vi "Migrate Measurement Dependencies.vi"(0 "project path":path, 1 "init":T1[](array[typedef]), 5 "measurement path":path, 7 "dependencies path":path[](array[path]), 9 "plug-in name":string, 11 "error in":errorcluster) -> (4 "project reference":refnum<vi>, 6 "measurement core reference":refnum<vi>, 8 "outside items":string[](array[string]), 10 "copied standalone VIs":cluster{"Lib path":path, "VI path":path}[](array[cluster]), 15 "error out":errorcluster)   [LabVIEW 2021, in "Multiple Converter.lvlib"]
uses:
  Multiple Converter.lvlib
  TypeDefs/Library Info.ctl
  Path Functions/Path Functions.lvlib
  Converter Reusables/Converter Reusables.lvlib
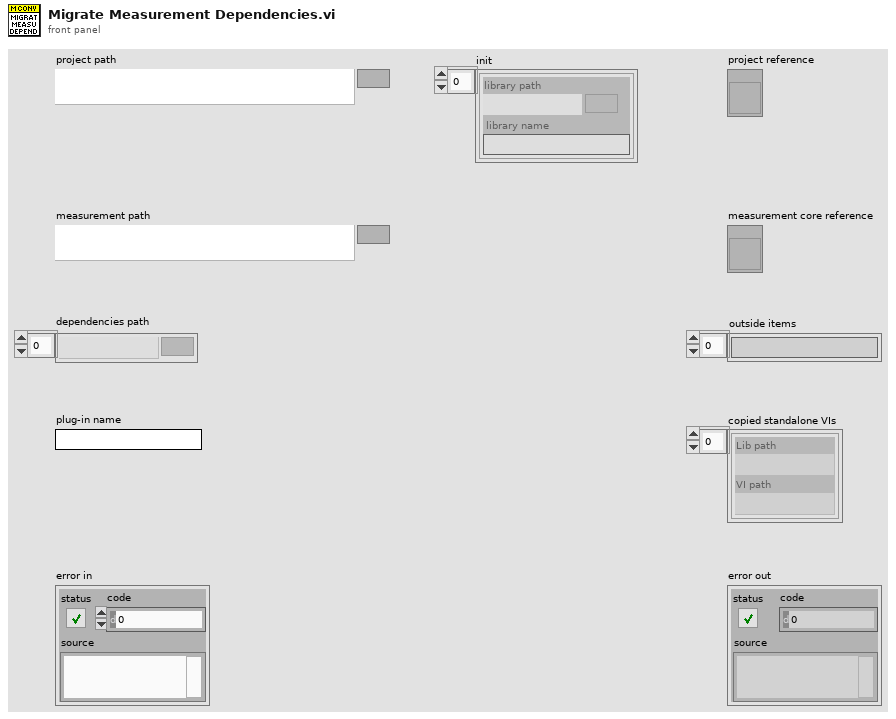
[diagram p1: front panel]
types:
  T1 = typedef "Multiple Converter.lvlib/Library Info.ctl" = cluster{"library path":path, "library name":string}
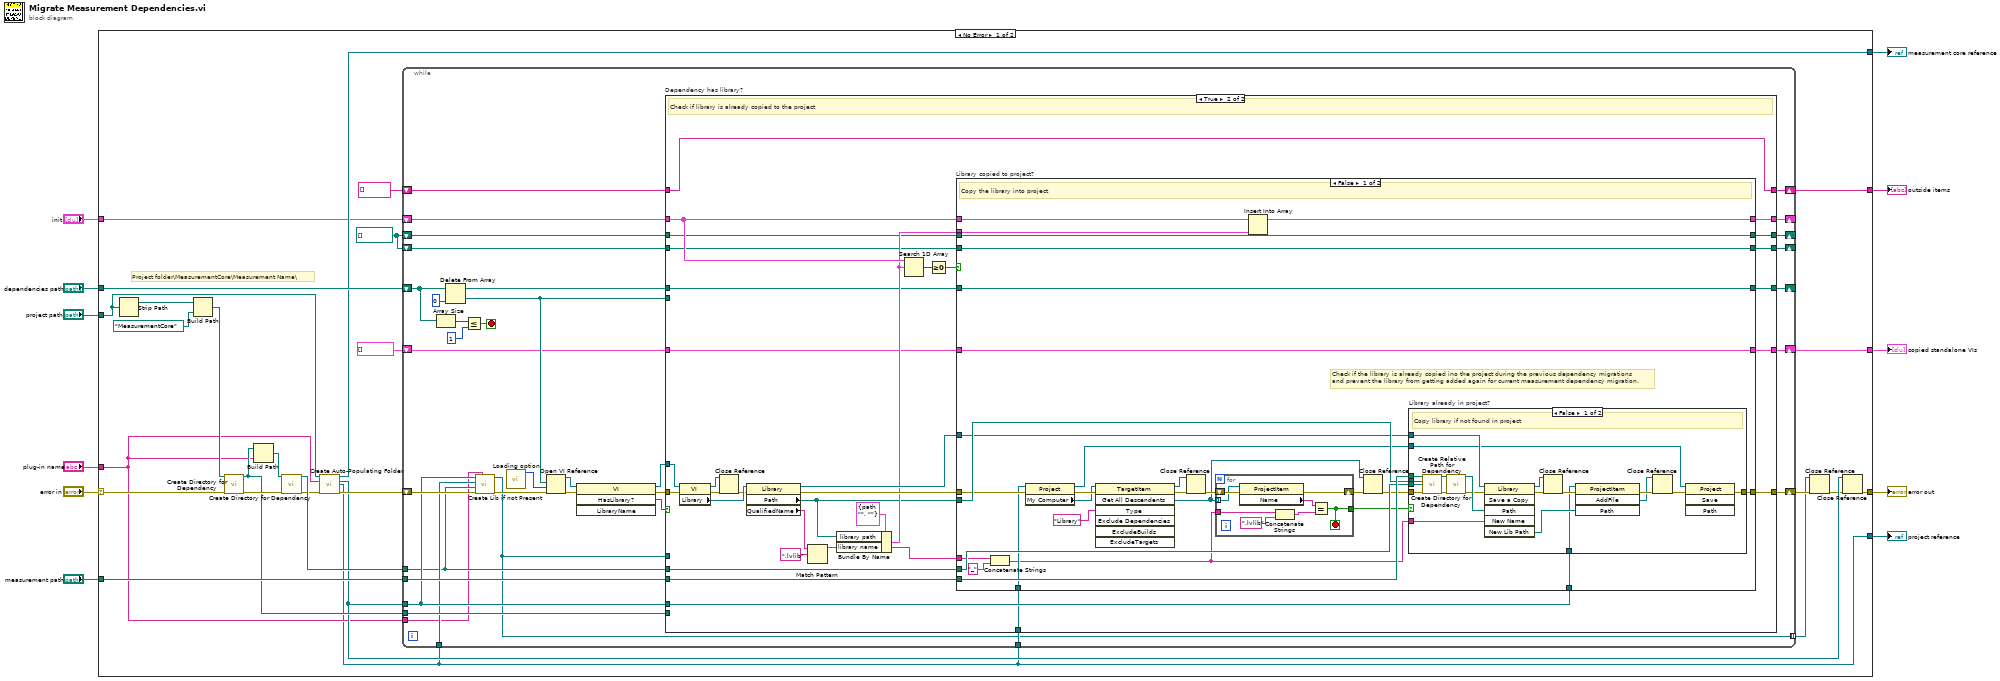
[diagram p0: block diagram]
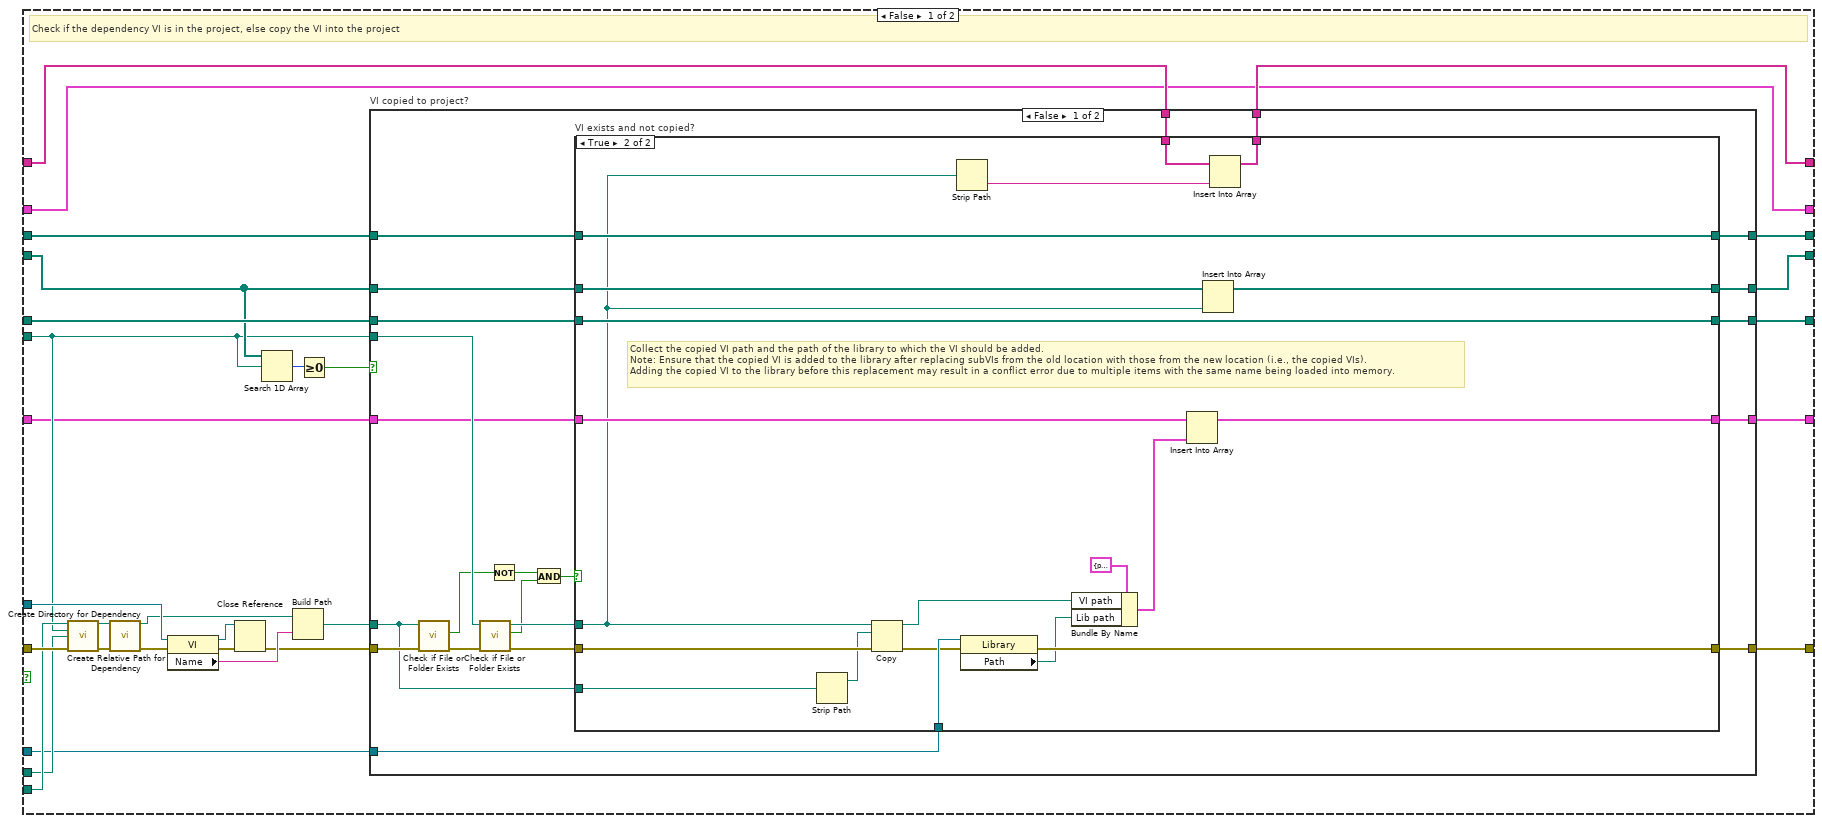
[diagram p2: hidden frame]
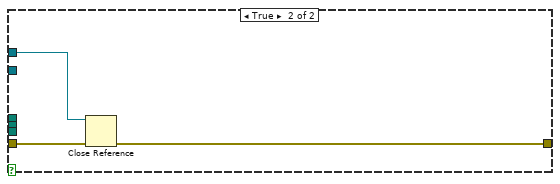
[diagram p5: hidden frame]
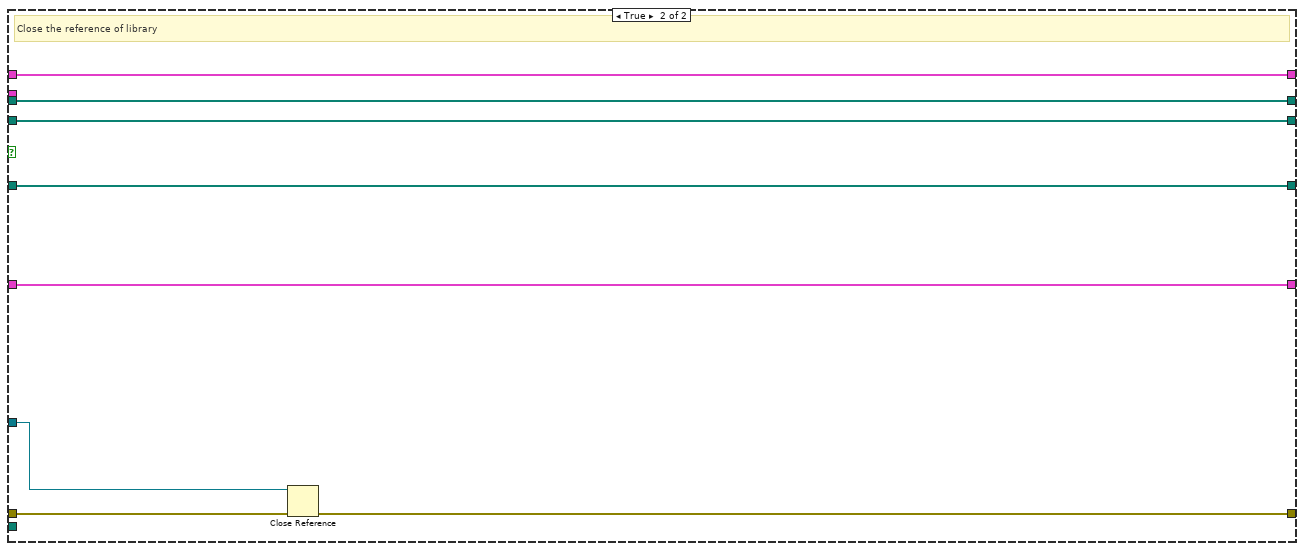
[diagram p6: hidden frame]
diagram:
  n1 = case shown="No Error" "error in" {
    selector: "error in" -> [w30 w257]
    tunnel: [w23 w257] -> w10
    tunnel: "project path" -> [w29 _]
    tunnel: "measurement path" -> [w34 _]
    tunnel: "dependencies path" -> [w38 _]
    tunnel: "plug-in name" -> [w21 _]
    tunnel: [w25 _] -> w5
    tunnel: [w18 _] -> w4
    tunnel: [w19 _] -> w3
    tunnel: "init" -> [w14 _]
    tunnel: [w12 _] -> w1
    frame No Error {
      w15 = path[] []
      # "Project folder\\MeasurementCore\\Measurement Name\\"
      n2 = Strip Path(path=w29) -> (stripped path=w33:path)  [unwired: 1 out]
      n3 = Build Path(base path=w33, name or relative path=path "MeasurementCore") -> (appended path=w31:path)
      n4 = call "Create Directory for Dependency.vi"("directory path"=w31, "error in"=w30) -> ("directory path out"=w24:path, "error out"=w28:errorcluster)  [unwired: 12 in]
      n5 = Build Path(base path=w24, name or relative path=w21) -> (appended path=w37:path)
      n6 = call "Create Directory for Dependency.vi"("directory path"=w37, "error in"=w28) -> ("directory path out"=w36:path, "error out"=w27:errorcluster)  [unwired: 12 in]
      n7 = call "Create Auto-Populating Folder.vi"("project path"=w29, "plug-in name"=w21, "error in"=w27) -> ("measurement core reference"=w25:refnum<vi>, "folder reference"=w22:refnum<vi>, "project reference"=w18:refnum<vi>, "error out"=w26:errorcluster)  [unwired: 9 in]
      n8 = while {
        shift-right: [w63] -> w35
        shift-left: w26 -> [w52]
        shift-right: [w56] -> _
        shift-left: w38 -> [w72]
        tunnel: w36 -> [w48]
        shift-right: [w62] -> _
        shift-left: w14 -> [w65]
        tunnel: w34 -> [w61]
        shift-right: [w58] -> _
        shift-left: w15 -> [w59]
        tunnel: w24 -> [w55]
        tunnel: w22 -> [w50]
        tunnel: w21 -> [w47]
        shift-right: [w53] -> w19
        shift-left: string[] [] -> [w54]
        tunnel: w18 -> [w49]
        tunnel: w18 -> [w46]
        shift-right: [w45] -> _
        shift-left: w15 -> [w44]
        tunnel: [w43] -> w16 mode=indexing
        shift-right: [w41] -> w12
        shift-left: cluster{"Lib path":path, "VI path":path}[] [] -> [w42]
        stop <- w71 stop-if-true
        n9 = Array Size(array=w72) -> (size(s)=w73:i32)
        n10 = Delete From Array(array=w72, index=0) -> (deleted portion=w60:path, array with subset deleted=w57:path[])  [unwired: 1 in]
        n11 = Less Or Equal?(x=w73, y=1) -> (x <= y?=w71:bool)
        n12 = call "Create Lib if not Present.vi"("plug-in name"=w47, "error in"=w52, "dest directory"=w48, "project ref"=w49, "virtual folder ref"=w50) -> ("error out"=w51:errorcluster, "library refnum"=w43:refnum<vi>)  [unwired: 5 in]
        n13 = call "Loading option.vi"() -> ("options"=w39:i32)  [unwired: 11 in]
        n14 = Open VI Reference(vi path=w60, options=w39, error in (no error)=w51) -> (vi reference=w69:refnum<vi>, error out=w70:errorcluster)  [unwired: 3 in]
        n15 = invoke class="VI" method="HasLibrary?"(reference=w69, error in=w70) -> (reference out=w66:refnum<vi>, error out=w67:errorcluster, "Has Library?"=w68:bool)  [unwired: 2 in, 1 out]
        n16 = case "Dependency has library?" shown="True" w68 {
          tunnel: w67 -> [w101 w187]
          tunnel: w66 -> [w97 w188]
          tunnel: w65 -> [w79 w175]
          tunnel: [w92 w176] -> w63
          tunnel: [w79 w174] -> w62
          tunnel: w61 -> [w100 w172]
          tunnel: w48 -> [w84 w170]
          tunnel: w60 -> [w87 _]
          tunnel: w59 -> [w88 w167]
          tunnel: [w83 w166] -> w58
          tunnel: w57 -> [w91 w165]
          tunnel: [w90 w164] -> w56
          tunnel: w55 -> [_ _]
          tunnel: w50 -> [_ w163]
          tunnel: w54 -> [w81 w162]
          tunnel: [w80 w162] -> w53
          tunnel: w43 -> [w82 _]
          tunnel: w46 -> [_ w161]
          tunnel: [w78 w159] -> w45
          tunnel: w44 -> [w77 w160]
          tunnel: w42 -> [w76 w158]
          tunnel: [w75 w157] -> w41
          frame False {
            # "Check if the dependency VI is in the project, else copy the VI into the project"
            n17 = call "Create Relative Path for Dependency.vi"("old main path"=w100, "old dependency path"=w87, "new dir"=w84, "error in"=w101) -> ("directory"=w99:path, "error out"=w102:errorcluster)  [unwired: 10 in]
            n18 = call "Create Directory for Dependency.vi"("directory path"=w99, "error in"=w102) -> ("directory path out"=w89:path, "error out"=w98:errorcluster)  [unwired: 12 in]
            n19 = property class="VI"(reference=w97, error in=w98) -> (reference out=w93:refnum<vi>, error out=w96:errorcluster, "Name"=w95:string)
            n20 = Close Reference(reference=w93, error in (no error)=w96) -> (error out=w94:errorcluster)
            n21 = Search 1D Array(1D array=w88, element=w87) -> (index of element=w86:i32)  [unwired: 1 in]
            n22 = Build Path(base path=w89, name or relative path=w95) -> (appended path=w74:path)
            n23 = Greater Or Equal To 0?(x=w86) -> (x >= 0?=w85:bool)
            n24 = case "VI copied to project?" shown="False" w85 {
              tunnel: w94 -> [w104 w156]
              tunnel: w87 -> [w124 _]
              tunnel: [w121 w156] -> w92
              tunnel: w88 -> [w120 w155]
              tunnel: [w119 w155] -> w83
              tunnel: w91 -> [w118 w154]
              tunnel: [w117 w154] -> w90
              tunnel: w81 -> [w111 w153]
              tunnel: [w110 w153] -> w80
              tunnel: w82 -> [w105 _]
              tunnel: [w109 w152] -> w78
              tunnel: w77 -> [w108 w152]
              tunnel: w76 -> [w107 w151]
              tunnel: [w106 w151] -> w75
              tunnel: w74 -> [w103 _]
              frame False {
                n25 = call <vilib>:"Check if File or Folder Exists.vi"("error in (no error)"=w104, "path"=w103) -> ("error out"=w116:errorcluster, "file or folder exists?"=w115:bool)  [unwired: 7 in, 1 out]
                n26 = call <vilib>:"Check if File or Folder Exists.vi"("error in (no error)"=w116, "path"=w124) -> ("error out"=w123:errorcluster, "file or folder exists?"=w113:bool, "dup path"=w122:path)  [unwired: 7 in]
                n27 = Not(x=w115) -> (.not. x?=w114:bool)
                n28 = And(x=w114, y=w113) -> (x .and. y?=w112:bool)
                n29 = case "VI exists and not copied?" shown="True" w112 {
                  tunnel: w123 -> [w130 w150]
                  tunnel: w122 -> [_ w131]
                  tunnel: [w130 w142] -> w121
                  tunnel: w120 -> [w129 w133]
                  tunnel: [w129 w132] -> w119
                  tunnel: w103 -> [_ w148]
                  tunnel: w118 -> [w128 w141]
                  tunnel: [w128 w141] -> w117
                  tunnel: w111 -> [w127 w147]
                  tunnel: [w127 w145] -> w110
                  tunnel: w105 -> [_ w144]
                  tunnel: [w126 w143] -> w109
                  tunnel: w108 -> [w126 w143]
                  tunnel: w107 -> [w125 w139]
                  tunnel: [w125 w138] -> w106
                  frame False {
                  }
                  frame True {
                    # "Collect the copied VI path and the path of the library to which the VI should be added.\nNote: Ensure that the copied VI is added to the library after replacing subVIs from the old location with those from the new location (i.e., the copied VIs).\nAdding the copied VI to the library before this replacement may result in a conflict error due to multiple items with the same name being loaded into memory."
                    n30 = Strip Path(path=w148) -> (stripped path=w149:path)  [unwired: 1 out]
                    n31 = Copy(8:w150, 10:w149, 11:w131) -> (0:w140:errorcluster, 3:w134:path)  [unwired: 2 in, 1 out]
                    n32 = Strip Path(path=w131) -> (name=w146:string)  [unwired: 1 out]
                    n33 = property class="Library"(reference=w144, error in=w140) -> (error out=w142:errorcluster, "Path"=w136:path)  [unwired: 1 out]
                    n34 = Bundle By Name(cluster=cluster{"Lib path":path, "VI path":path} {"Lib path"=path "", "VI path"=path ""}, "VI path"=w134, "Lib path"=w136) -> (w135:cluster{"Lib path":path, "VI path":path})
                    n35 = Insert Into Array(array=w139, new element=w135) -> (w138:cluster{"Lib path":path, "VI path":path}[])  [unwired: 1 in]
                    n36 = Insert Into Array(array=w133, new element=w131) -> (w132:path[])  [unwired: 1 in]
                    n37 = Insert Into Array(array=w147, new element=w146) -> (w145:string[])  [unwired: 1 in]
                  }
                }
              }
              frame True {
              }
            }
          }
          frame True {
            # "Check if library is already copied to the project"
            n38 = property class="VI"(reference=w188, error in=w187) -> (reference out=w178:refnum<vi>, error out=w186:errorcluster, "Library"=w185:refnum<vi>)
            n39 = Close Reference(reference=w178, error in (no error)=w186) -> (error out=w179:errorcluster)
            n40 = property class="Library"(reference=w185, error in=w179) -> (reference out=w177:refnum<vi>, error out=w180:errorcluster, "Path"=w171:path, "QualifiedName"=w181:string)
            n41 = Match Pattern(string=w181, regular expression=".lvlib") -> (before substring=w168:string)  [unwired: 1 in, 3 out]
            n42 = Bundle By Name(cluster=T1 {"library path"=path "", "library name"=""} ("Cluster"), "library path"=w171, "library name"=w168) -> (w173:T1)
            n43 = Search 1D Array(1D array=w175, element=w173) -> (index of element=w183:i32)  [unwired: 1 in]
            n44 = Greater Or Equal To 0?(x=w183) -> (x >= 0?=w182:bool)
            n45 = case "Library copied to project?" shown="False" w182 {
              tunnel: w180 -> [w203 w255]
              tunnel: w177 -> [w211 w256]
              tunnel: [w205 w254] -> w176
              tunnel: w175 -> [w217 w253]
              tunnel: [w216 w253] -> w174
              tunnel: w173 -> [w215 _]
              tunnel: w172 -> [w214 _]
              tunnel: w171 -> [w213 _]
              tunnel: w170 -> [w212 _]
              tunnel: w168 -> [w207 _]
              tunnel: w167 -> [w210 w252]
              tunnel: [w210 w252] -> w166
              tunnel: [w209 w251] -> w164
              tunnel: w165 -> [w209 w251]
              tunnel: w163 -> [w208 _]
              tunnel: w161 -> [w202 _]
              tunnel: [w204 w250] -> w159
              tunnel: w160 -> [w204 w250]
              tunnel: w158 -> [w190 w249]
              tunnel: [w190 w249] -> w157
              frame False {
                # "Check if the library is already copied ino the project during the previous dependency migrations \nand prevent the library from getting added again for current measurement dependency migration."
                # "Copy the library into project"
                n46 = Concatenate Strings(w207, "_" ("string")) -> (w189:string)
                n47 = property class="Project"(reference=w202, error in=w203) -> (reference out=w199:refnum<vi>, error out=w201:errorcluster, "My Computer"=w200:refnum<vi>)
                n48 = invoke class="TargetItem" method="Get All Descendents"(reference=w200, error in=w201, "Type"="Library") -> (reference out=w195:refnum<vi>, error out=w197:errorcluster, "All Descendents"=w192:refnum<vi>[])  [unwired: 4 in, 4 out]
                n49 = Close Reference(reference=w195, error in (no error)=w197) -> (error out=w196:errorcluster)
                n50 = for {
                  shift-right: [w247] -> w194
                  shift-left: w196 -> [w248]
                  tunnel: w192 -> [w246] mode=indexing
                  tunnel: w189 -> [w241]
                  tunnel: [w244] -> w191
                  stop <- w244 stop-if-true
                  n51 = property class="ProjectItem"(reference=w246, error in=w248) -> (error out=w247:errorcluster, "Name"=w245:string)  [unwired: 1 out]
                  n52 = Concatenate Strings(w241, ".lvlib" ("string")) -> (w242:string)
                  n53 = Equal?(x=w245, y=w242) -> (x = y?=w244:bool)
                }
                n54 = Insert Into Array(array=w217, new element=w215) -> (w216:T1[])  [unwired: 1 in]
                n55 = Close Reference(reference=w192, error in (no error)=w194) -> (error out=w193:errorcluster)
                n56 = case "Library already in project?" shown="False" w191 {
                  tunnel: w214 -> [w235 _]
                  tunnel: w213 -> [w234 _]
                  tunnel: w212 -> [w233 _]
                  tunnel: w211 -> [w229 w238]
                  tunnel: w208 -> [w222 _]
                  tunnel: [w221 w239] -> w205
                  tunnel: w199 -> [w220 _]
                  tunnel: w189 -> [w219 _]
                  tunnel: w193 -> [w218 w240]
                  frame False {
                    # "Copy library if not found in project"
                    n57 = call "Create Relative Path for Dependency.vi"("old main path"=w235, "old dependency path"=w234, "new dir"=w233, "error in"=w218) -> ("directory"=w231:path, "error out"=w232:errorcluster)  [unwired: 10 in]
                    n58 = call "Create Directory for Dependency.vi"("directory path"=w231, "error in"=w232) -> ("directory path out"=w230:path, "error out"=w228:errorcluster)  [unwired: 12 in]
                    n59 = invoke class="Library" method="Save a Copy"(reference=w229, error in=w228, "Path"=w230, "New Name"=w219) -> (reference out=w236:refnum<vi>, error out=w237:errorcluster, "New Lib Path"=w225:path)  [unwired: 2 in, 3 out]
                    n60 = Close Reference(reference=w236, error in (no error)=w237) -> (error out=w227:errorcluster)
                    n61 = invoke class="ProjectItem" method="AddFile"(reference=w222, error in=w227, "Path"=w225) -> (error out=w226:errorcluster, "AddFile"=w223:refnum<vi>)  [unwired: 1 in, 2 out]
                    n62 = Close Reference(reference=w223, error in (no error)=w226) -> (error out=w224:errorcluster)
                    n63 = invoke class="Project" method="Save"(reference=w220, error in=w224) -> (error out=w221:errorcluster)  [unwired: 2 in, 3 out]
                  }
                  frame True {
                    n64 = Close Reference(reference=w238, error in (no error)=w240) -> (error out=w239:errorcluster)
                  }
                }
              }
              frame True {
                # "Close the reference of library"
                n65 = Close Reference(reference=w256, error in (no error)=w255) -> (error out=w254:errorcluster)
              }
            }
          }
        }
      }
      n66 = Close Reference(reference=w16, error in (no error)=w35) -> (error out=w17:errorcluster)
      n67 = Close Reference(reference=w22, error in (no error)=w17) -> (error out=w23:errorcluster)
    }
    frame Error {
    }
  }
  "error out" <- w10
  "measurement core reference" <- w5
  "project reference" <- w4
  "outside items" <- w3
  "copied standalone VIs" <- w1
